vi "Verify Mock.vi"(8 "error in (no error)":errorcluster, 11 "Mock In":refnum<class "LMock Mock.lvclass">) -> (0 "error out":errorcluster, 1 "Errors":errorcluster[](array[cluster]), 2 "Results":cluster{"Passed?":bool, "Message":string}[](array[cluster]))   [LabVIEW 2020, in "LMock Mock.lvclass"]
uses:
  LMock Mock.lvclass
  LMock Mock.lvclass/LMock Mock.ctl
  Core/Expectation/Expectation.lvclass
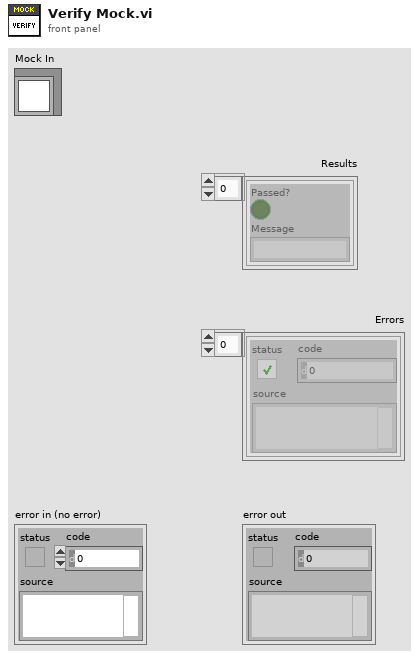
[diagram p1: front panel]
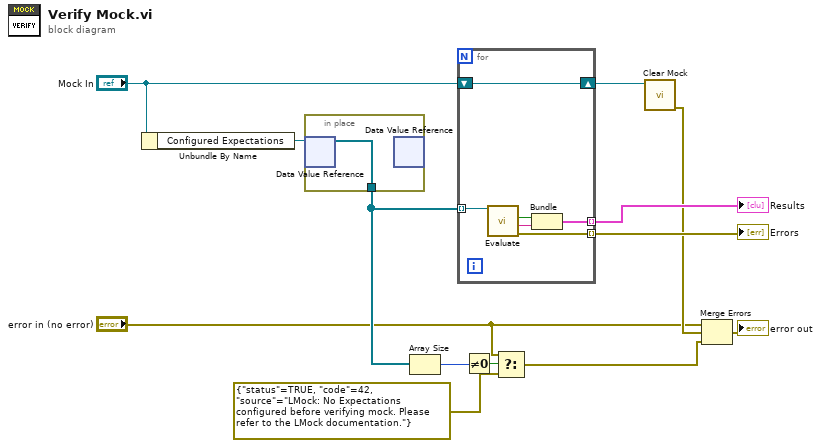
[diagram p0: block diagram]
diagram:
  n1 = Unbundle By Name("Mock In") -> ("Configured Expectations"=w11:refnum<data-value>)
  n2 = in-place {
    in-place-border: [w14] -> w6
    n3 = in-place-dvr #1(w11) -> (w14:refnum<class "Expectation.lvclass">[])  [unwired: 1 out]
    n4 = in-place-dvr #1() -> ()  [unwired: 1 in, 2 out]
  }
  n5 = Array Size(array=w6) -> (size(s)=w4:i32)
  n6 = for {
    tunnel: [w20] -> w13 mode=indexing
    tunnel: w6 -> [w19] mode=indexing
    tunnel: [w16] -> w12 mode=indexing
    shift-right: [w15] -> w7
    shift-left: "Mock In" -> [w15]
    n7 = call-dynamic "Evaluate.vi"("Expectation in"=w19) -> ("error out"=w20:errorcluster, "Message"=w17:string, "Passed?"=w18:bool)  [unwired: 8 in]
    n8 = Bundle("Passed?"=w18, "Message"=w17) -> (w16:cluster{"Passed?":bool, "Message":string})  [unwired: 1 in]
  }
  "Errors" <- w13
  "Results" <- w12
  n9 = Not Equal To 0?(x=w4) -> (x != 0?=w5:bool)
  n10 = Select(t="error in (no error)", s=w5, f=errorcluster {"status"=TRUE, "code"=42, "source"="LMock: No Expectations configured before verifying mock. Please refer to the LMock documentation."}) -> (s? t:f=w2:errorcluster)
  n11 = call-dynamic "Clear Mock.vi"("Mock In"=w7) -> ("error out"=w10:errorcluster)  [unwired: 10 in]
  n12 = Merge Errors("error in (no error)", w10, w2) -> (→"error out":errorcluster)
